vi "Load VI Into Memory.vi"(8 "error in (no error)":errorcluster, 10 "VI Path":path, 11 "Session in":refnum<class "Session.lvclass">) -> (0 "error out":errorcluster, 3 "Session out":refnum<class "Session.lvclass">)   [LabVIEW 2020, in "Save for Previous Version.lvlib" / "Session.lvclass"]
uses:
  Session.lvclass
  VI File/VI File.lvclass
  Session.lvclass/Session.ctl
  <userlib>/_OpenG.lib/file/file.llb/Append Path to Root if Relative - Scalar__ogtk.vi
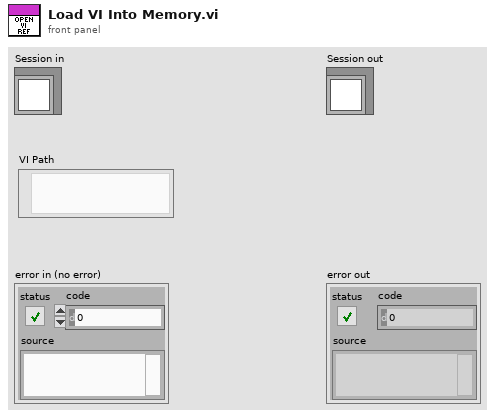
[diagram p1: front panel]
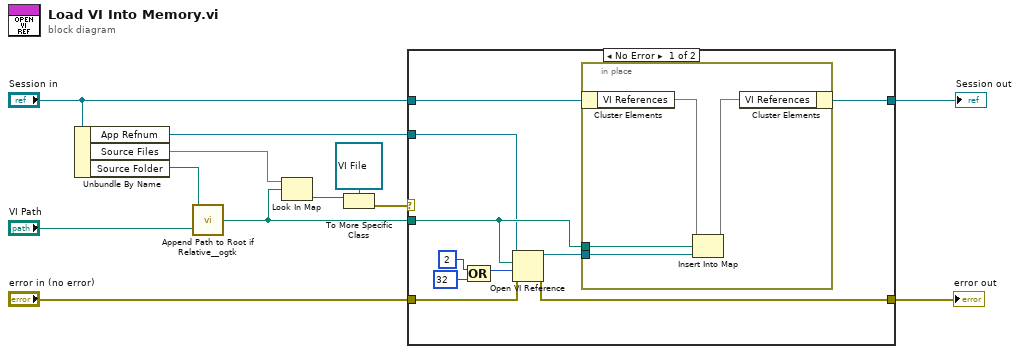
[diagram p0: block diagram]
diagram:
  n1 = Unbundle By Name("Session in") -> ("App Refnum"=w1:refnum<vi>, "Source Files"=w6:map{path, refnum<class "File.lvclass">}, "Source Folder"=w8:path)
  n2 = call-poly <userlib>:"Append Path to Root if Relative__ogtk.vi"("Absolute or Relative Path"="VI Path", "Root Path"=w8) -> ("Absolute or Appended Path"=w5:path)
  n3 = Look In Map(map=w6, key=w5) -> (value=w3:refnum<class "File.lvclass">)  [unwired: 1 in, 1 out]
  n4 = To More Specific Class(target class=refnum<class "VI File.lvclass"> refnum ("Save for Previous Version.lvlib:VI File.lvclass"), reference=w3) -> (error out=w2:errorcluster)  [unwired: 1 in, 1 out]
  n5 = case shown="No Error" w2 {
    tunnel: [w22 w28] -> w12
    tunnel: [w17 w27] -> w11
    tunnel: "error in (no error)" -> [w16 w27]
    tunnel: "Session in" -> [w15 w28]
    tunnel: w5 -> [w14 _]
    tunnel: w1 -> [w13 _]
    frame No Error {
      n6 = Compound Arithmetic op=OR(2 ("options"), 32 ("options")) -> (w20:i32)
      n7 = Open VI Reference(application reference (local)=w13, vi path=w14, options=w20, error in (no error)=w16) -> (vi reference=w21:refnum<vi>, error out=w17:errorcluster)  [unwired: 2 in]
      n8 = in-place {
        in-place-border: w14 -> [w24]
        in-place-border: w21 -> [w23]
        n9 = in-place-cluster #1(w15) -> ("VI References"=w26:map{path, refnum<vi>})
        n10 = Insert Into Map(map in=w26, key=w24, value=w23) -> (map out=w25:map{path, refnum<vi>})  [unwired: 2 out]
        n11 = in-place-cluster #1("VI References"=w25) -> (w22:refnum<class "Session.lvclass">)
      }
    }
    frame Error {
    }
  }
  "Session out" <- w12
  "error out" <- w11
